vi "Write OD Var Status.vi"(8 "error in (no error)":errorcluster, 10 "OD Var Status":i32[](array[numeric]), 11 "OD Batch in":refnum<class "OD Batch.lvclass">) -> (0 "error out":errorcluster, 3 "OD Batch out":refnum<class "OD Batch.lvclass">)   [LabVIEW 2023, in "xnet_canopen.lvlib" / "OD Batch.lvclass"]
uses:
  OD Batch.lvclass
  OD Batch.lvclass/OD Batch.ctl
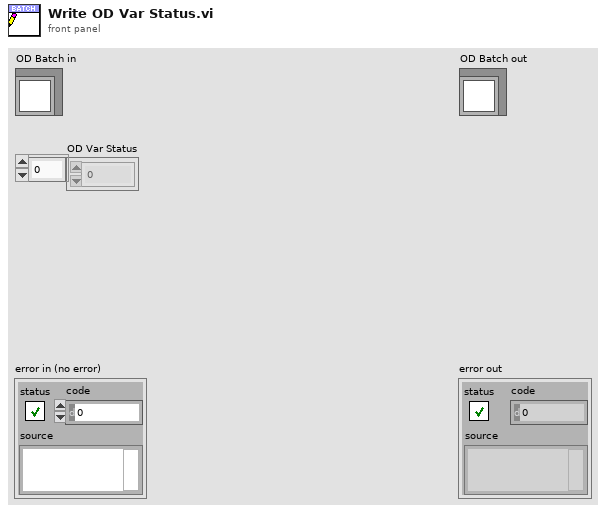
[diagram p1: front panel]
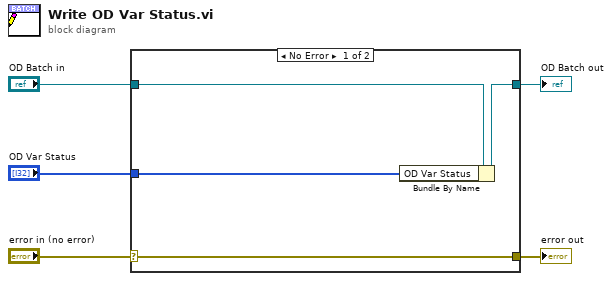
[diagram p0: block diagram]
diagram:
  n1 = case shown="No Error" "error in (no error)" {
    selector: "error in (no error)" -> [w9 w10]
    tunnel: [w9 w10] -> w4
    tunnel: [w7 w11] -> w2
    tunnel: "OD Batch in" -> [w8 w11]
    tunnel: "OD Var Status" -> [w6 _]
    frame No Error {
      n2 = Bundle By Name(cluster=w8, "OD Var Status"=w6) -> (w7:refnum<class "OD Batch.lvclass">)
    }
    frame Error {
    }
  }
  "error out" <- w4
  "OD Batch out" <- w2
